vi "Ignition Main.vi"(8 "error in":errorcluster, 9 "URL":string, 10 "folder name":string="NonUDT", 11 "Sequence Context":refnum<k7>) -> (0 "error out":errorcluster)   [LabVIEW 2025]
uses:
  Ignition Tx.ctl
  <vilib>/OPCUA/client/Connect2.vi
  <vilib>/OPCUA/NI OPC UA Client.lvlib
panel:
  out "Tester Tx":T1
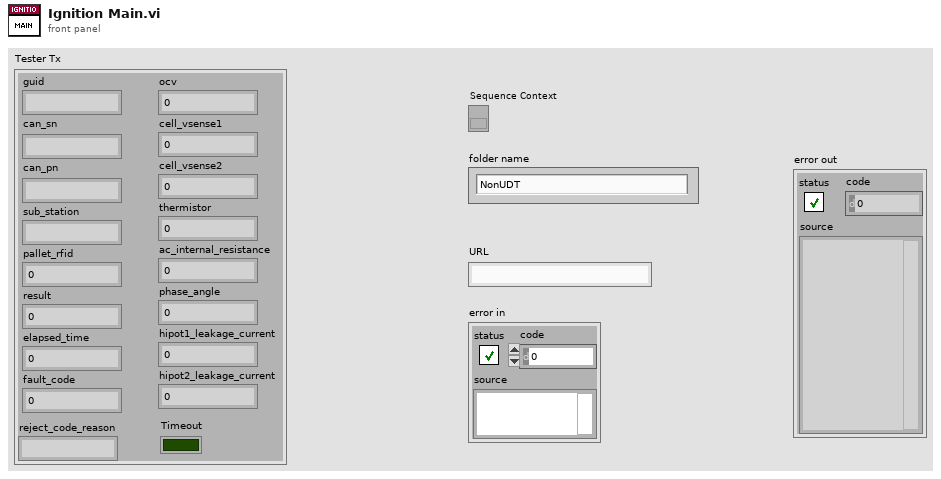
[diagram p1: front panel]
types:
  T1 = typedef "Ignition Tx.ctl" = cluster{"thermistor":dbl, "phase_angle":dbl, "pallet_rfid":dbl, "ocv":dbl, "cell_vsense1":dbl, "cell_vsense2":dbl, "hipot1_leakage_current":dbl, "hipot2_leakage_current":dbl, "guid":string, "can_sn":string, "can_pn":string, "ac_internal_resistance":dbl, "sub_station":string, "fault_code":i32, "elapsed_time":i32, "result":i32, "reject_code_reason":string, "Timeout":bool}
  T2 = typedef "Submodule EOL.lvlib/Ignition Tx.ctl" = cluster{"thermistor":dbl, "phase_angle":dbl, "pallet_rfid":dbl, "ocv":dbl, "cell_vsense1":dbl, "cell_vsense2":dbl, "hipot1_leakage_current":dbl, "hipot2_leakage_current":dbl, "guid":string, "can_sn":string, "can_pn":string, "ac_internal_resistance":dbl, "sub_station":string, "fault_code":i32, "elapsed_time":i32, "result":i32, "reject_code_reason":string, "Timeout":bool}
  T3 = typedef "OPC UA Client Refnum.ctl" = refnum<k21>
  T4 = typedef "Subscription ID.ctl" = u32
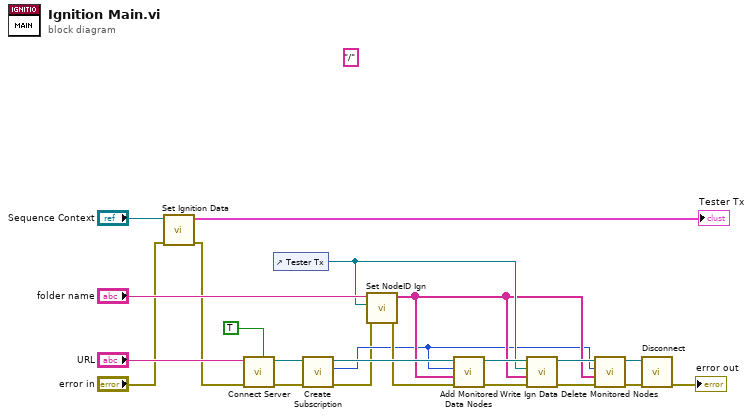
[diagram p0: block diagram]
diagram:
  (unwired) "/" ("Deliminated Char")
  n1 = call "Set Ignition Data.vi"("error in"="error in", "Sequence Context"="Sequence Context") -> ("error out"=w2:errorcluster, "Ignition Tx out"=→"Tester Tx":T2)  [unwired: 8 in]
  n2 = call-poly <vilib>:"Connect Server.vi"("trust any server (F)"=TRUE, "error in (no error)"=w2, "server endpoint URL"="URL") -> ("error out"=w22:errorcluster, "OPC UA client refnum out"=w21:T3)  [unwired: 6 in, 1 out]
  n3 = control-ref of="Tester Tx"() -> (w11:refnum<vi>)
  n4 = call <vilib>:"Create Subscription.vi"("error in (no error)"=w22, "OPC UA client refnum in"=w21) -> ("error out"=w4:errorcluster, "subscription ID out"=w5:T4, "OPC UA client refnum out"=w18:T3)  [unwired: 5 in, 2 out]
  n5 = call "Set NodeID Ign.vi"("error in (no error)"=w4, "Tester Tx"=w11, "folder name"="folder name") -> ("error out"=w14:errorcluster, "NodeIDs"=w7:string[])  [unwired: 7 in]
  n6 = call <vilib>:"Add Monitored Data Nodes.vi"("error in (no error)"=w14, "node IDs"=w7, "subscription ID in"=w5, "OPC UA client refnum in"=w18) -> ("error out"=w13:errorcluster, "OPC UA client refnum out"=w12:T3)  [unwired: 4 in, 2 out]
  n7 = call "Write Ign Data.vi"("error in (no error)"=w13, "NodeIDs"=w7, "Control Ref"=w11, "OPC UA client refnum"=w12) -> ("error out"=w9:errorcluster, "OPC UA client refnum"=w10:T3)  [unwired: 6 in]
  n8 = call <vilib>:"Delete Monitored Nodes.vi"("error in (no error)"=w9, "node IDs"=w7, "subscription ID in"=w5, "OPC UA client refnum in"=w10) -> ("error out"=w8:errorcluster, "OPC UA client refnum out"=w6:T3)  [unwired: 3 in, 3 out]
  n9 = call <vilib>:"Disconnect.vi"("error in (no error)"=w8, "OPC UA client refnum in"=w6) -> ("error out"=→"error out":errorcluster)  [unwired: 9 in]
